vi "tof.vi"(10 "Time":i32, 11 "START in":bool) -> (2 "ET 4":i32, 3 "Q 4":bool)   [LabVIEW 2020]
panel:
  out "Time 2":i32
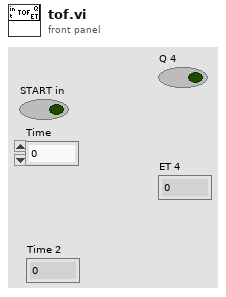
[diagram p1: front panel]
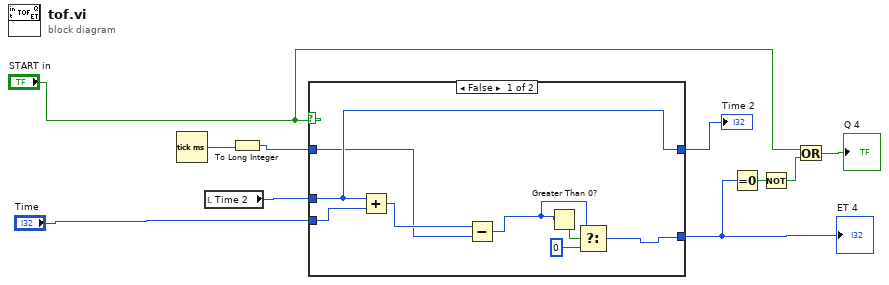
[diagram p0: block diagram]
diagram:
  n1 = Tick Count (ms)() -> (millisecond timer value=w6:u32)
  n2 = local read "Time 2"() -> (w2:i32)
  n3 = To Long Integer(number=w6) -> (32bit integer=w7:i32)
  n4 = case shown="False" "START in" {
    tunnel: w7 -> [w12 w20]
    tunnel: [w13 w20] -> w1
    tunnel: w2 -> [w13 _]
    tunnel: "Time" -> [w14 w19]
    tunnel: [w11 w19] -> w8
    frame False {
      n5 = Add(x=w13, y=w14) -> (x+y=w18:i32)
      n6 = Subtract(x=w18, y=w12) -> (x-y=w16:i32)
      n7 = Greater Than 0?(x=w16) -> (x > 0?=w17:bool)
      n8 = Select(t=w16, s=w17, f=0) -> (s? t:f=w11:i32)
    }
    frame True {
    }
  }
  "ET 4" <- w8
  "Time 2" <- w1
  n9 = Equal To 0?(x=w8) -> (x = 0?=w9:bool)
  n10 = Not(x=w9) -> (.not. x?=w10:bool)
  n11 = Or(x="START in", y=w10) -> (x .or. y?=→"Q 4":bool)
